vi "Call Function with I32 Python Objects.vi"(8 "error in (no error)":errorcluster) -> (0 "error out":errorcluster)   [LabVIEW 2020]
uses:
  908d8fb0-7b42-46e8-9e96-a0c6d44c2c93.vi
  G-Embedded-Python-Interpreter-Toolkit/Null Py Object Refnum.vi
  908d8fb0-7b42-46e8-9e96-a0c6d44c2c93.vi/96ddca92-7bbf-40e2-a1a5-d32f291eb6af.vi
  G-Embedded-Python-Interpreter-Toolkit/Pointer Sized Ref to Python Object Reference.vi
  G-Embedded-Python-Interpreter-Toolkit/Generate Argument Type Info.vi
  G-Embedded-Python-Interpreter-Toolkit/Python Object Reference to Pointer Sized Ref.vi
  G-Embedded-Python-Interpreter-Toolkit/Variant to Type Info.vi
  G-Embedded-Python-Interpreter-Toolkit/Bad Type Error.vi
  G-Embedded-Python-Interpreter-Toolkit/Variant to Type Info.vi/8cdebbe9-3e59-4fbe-97b0-695fa0ebc24d.vi
  G-Embedded-Python-Interpreter-Toolkit/Merge Call Library Errors.vi
  <vilib>/Utility/Data Type/Get Type Information.vi
  <vilib>/Utility/error.llb/Error Cluster From Error Code.vi
  <vilib>/Utility/Data Type/Get Array Information.vi
  <vilib>/Utility/Data Type/Get Cluster Information.vi
  <vilib>/addons/_JKI Toolkits/Caraya/classes/Assert/Assert Not Error.vi
  <vilib>/addons/_JKI Toolkits/Caraya/classes/Assert/Assert Equal Value and Type_Variant.vi
  <vilib>/Comparison/Equal/Equal Functor/Equal Functor.lvclass
  G-Embedded-Python-Interpreter-Toolkit/G-Embedded-Python-Interpreter-Toolkit.lvlib
  <vilib>/addons/_JKI Toolkits/Caraya/classes/Test/Test.lvclass
  <vilib>/addons/_JKI Toolkits/Caraya/classes/Assert/Assert.lvclass
panel:
  out "Value":i32
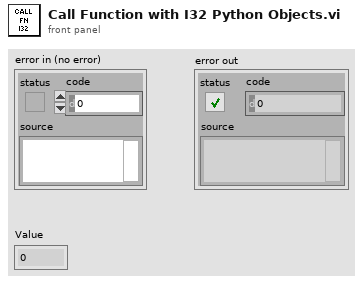
[diagram p1: front panel]
types:
  T1 = typedef "G-Embedded-Python-Interpreter-Toolkit.lvlib/Python Object Reference.ctl" = refnum<k1>
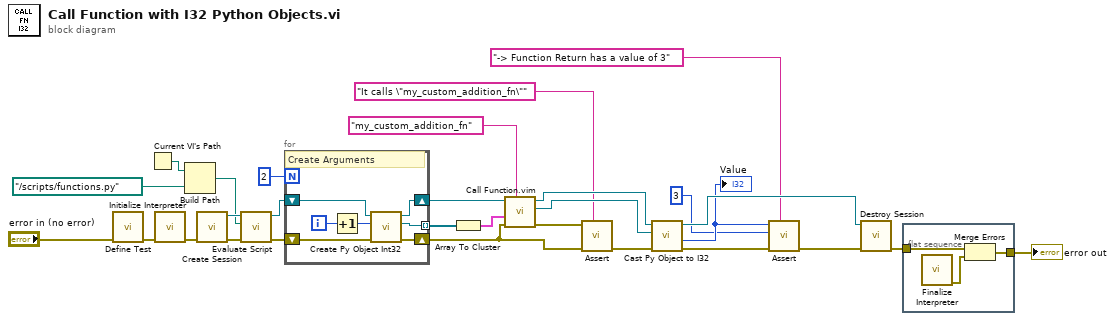
[diagram p0: block diagram]
diagram:
  n1 = call <vilib>:"Define Test.vi"("error in (no error)"="error in (no error)") -> ("error out"=w29:errorcluster)  [unwired: 10 in]
  n2 = Current VI's Path() -> (path=w24:path)
  n3 = call "Initialize Interpreter.vi"("error in (no error)"=w29) -> ("error out"=w26:errorcluster)  [unwired: 9 in, 1 out]
  n4 = Build Path(base path=w24, name or relative path=path "../scripts/functions.py" ("Path")) -> (appended path=w22:path)
  n5 = call "Create Session.vi"("error in (no error)"=w26) -> ("error out"=w21:errorcluster, "Session Handle"=w25:refnum<data-value>)  [unwired: 9 in]
  n6 = call "Evaluate Script.vi"("error in (no error)"=w21, "Script File Path"=w22, "Session Handle in"=w25) -> ("error out"=w18:errorcluster, "Session Handle out"=w19:refnum<data-value>)  [unwired: 7 in]
  n7 = for {
    N: 2 -> [_]
    shift-right: [w32] -> w17
    shift-left: w19 -> [w36]
    shift-right: [w33] -> w6
    shift-left: w18 -> [w35]
    tunnel: [w31] -> w16 mode=indexing
    i -> [w34]
    # "Create Arguments"
    n8 = Increment(x=w34) -> (x+1=w30:i32)
    n9 = call "Create Py Object Int32.vi"("error in (no error)"=w35, "Value"=w30, "Session Handle in"=w36) -> ("error out"=w33:errorcluster, "Python Object Refnum"=w31:T1, "Session Handle out"=w32:refnum<data-value>)  [unwired: 6 in]
  }
  n10 = Array To Cluster(array=w16) -> (cluster=w1:cluster{"[0]":T1, "[1]":T1})
  n11 = call "Call Function.vim"("Function Name"="my_custom_addition_fn", "error in (no error)"=w6, "Arguments in (Default - None)"=w1, "Data Value Reference in"=w17) -> ("error out"=w5:errorcluster, "Returned Python Object Refnum"=w14:T1, "Data Value Reference out"=w15:refnum<data-value>)  [unwired: 5 in]
  n12 = call-poly <vilib>:"Assert.vi"("Label"="It calls \"my_custom_addition_fn\"", "error in (no error)"=w6, "Not Error?"=w5) -> ("error out"=w4:errorcluster)  [unwired: 8 in]
  n13 = call "Cast Py Object to I32.vi"("error in (no error)"=w4, "Python Object Refnum in"=w14, "Session Handle in"=w15) -> ("error out"=w3:errorcluster, "Value"=w11:i32, "Session Handle out"=w13:refnum<data-value>)  [unwired: 5 in, 1 out]
  "Value" <- w11
  n14 = call-poly <vilib>:"Assert.vi"("Label"="-> Function Return has a value of 3", "error in (no error)"=w3, "Y"=3 ("Value"), "X"=w11) -> ("error out"=w10:errorcluster)  [unwired: 7 in]
  n15 = call "Destroy Session.vi"("error in (no error)"=w10, "Session Handle"=w13) -> ("error out"=w20:errorcluster)  [unwired: 9 in]
  n16 = flat-sequence {
    tunnel: w20 -> [w39]
    tunnel: [w37] -> w27
    frame #0 {
      n17 = call "Finalize Interpreter.vi"() -> ("error out"=w38:errorcluster)  [unwired: 11 in]
      n18 = Merge Errors(w39, w38) -> (w37:errorcluster)
    }
  }
  "error out" <- w27
